vi "Pass data using reference.vi"(11 "error in":errorcluster) -> (15 "error out":errorcluster)   [LabVIEW 2021, in "Voltage Measurement.lvlib"]
uses:
  MeasurementCore/controls/Voltage Config.ctl
  MeasurementCore/controls/Current Config.ctl
  8c08564a-52c5-40b6-a610-6b453a234e3b.vi
  ff7b3996-5054-42a4-b452-886b26c0f36c.vi
  8c08564a-52c5-40b6-a610-6b453a234e3b.vi/36c45d0c-28c4-4d78-84df-ca3969178567.vi
  ff7b3996-5054-42a4-b452-886b26c0f36c.vi/36c45d0c-28c4-4d78-84df-ca3969178567.vi
  8c08564a-52c5-40b6-a610-6b453a234e3b.vi/36c45d0c-28c4-4d78-84df-ca3969178567.vi/6651a77e-856e-4bcd-af5a-c0c13b264cc1.vi
  ff7b3996-5054-42a4-b452-886b26c0f36c.vi/36c45d0c-28c4-4d78-84df-ca3969178567.vi/6651a77e-856e-4bcd-af5a-c0c13b264cc1.vi
  <vilib>/JDP Science/JSONtext/JSON text to Variant.vi
  <vilib>/JDP Science/JSONtext/LVClass Serializer/JSONtext LVClass Serializer.lvclass
  Voltage Measurement.lvlib
  MeasurementCore/Main_Voltage Measurement.lvlib
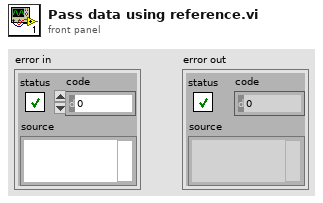
[diagram p1: front panel]
types:
  T1 = typedef "Main_Voltage Measurement.lvlib/Voltage Config.ctl" = cluster{"Voltage Level":dbl, "Voltage Level Range":dbl}
  T2 = typedef "Main_Voltage Measurement.lvlib/Current Config.ctl" = cluster{"Current Limit":dbl, "Current Limit Range":dbl}
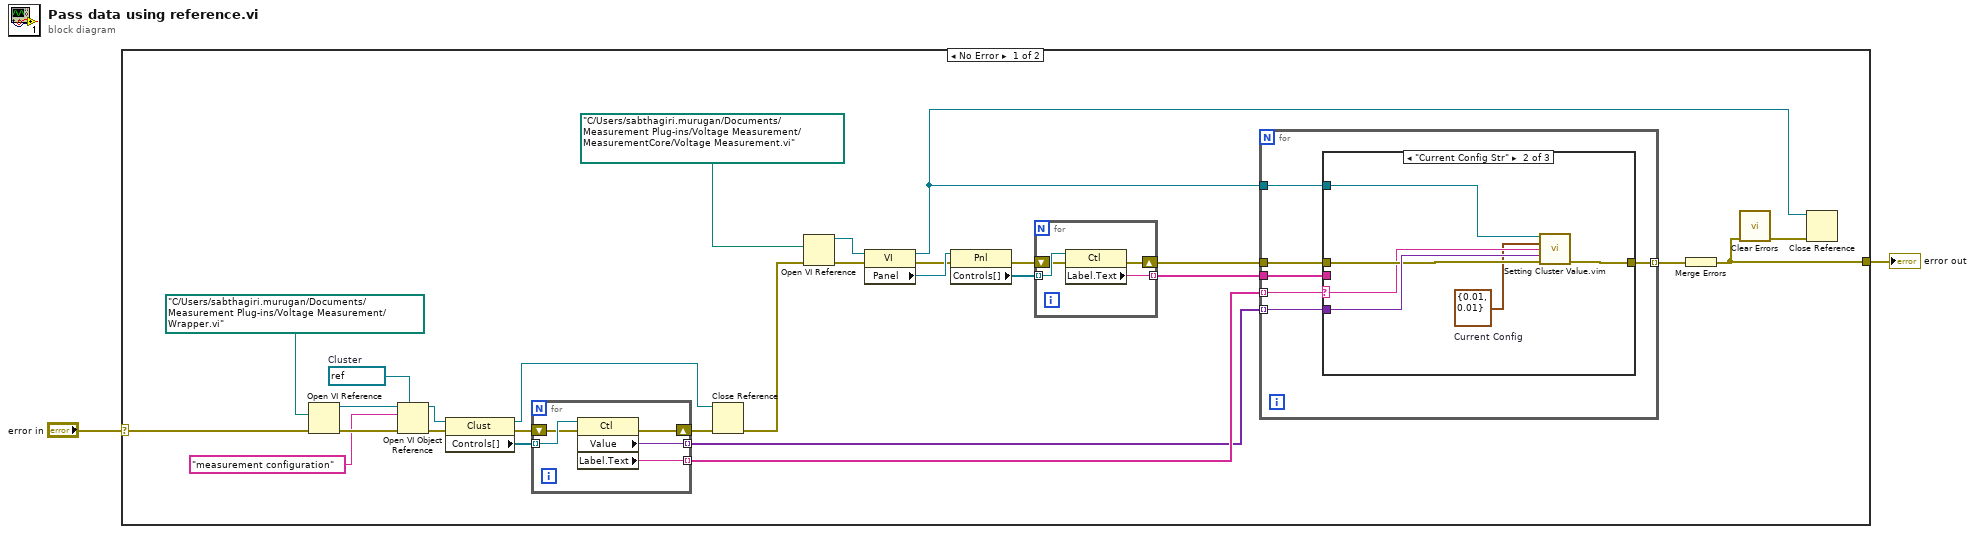
[diagram p0: block diagram]
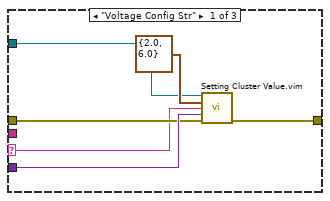
[diagram p2: hidden frame]
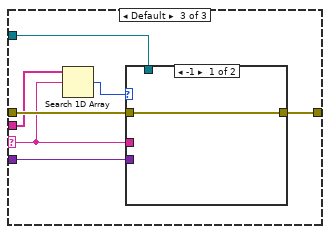
[diagram p3: hidden frame]
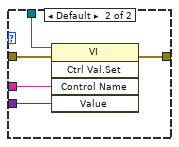
[diagram p4: hidden frame]
diagram:
  n1 = case shown="No Error" "error in" {
    selector: "error in" -> [w29 w71]
    tunnel: [w12 w71] -> w2
    frame No Error {
      w22 = refnum<vi> refnum  # Cluster
      n2 = Open VI Reference(vi path=path "C:/Users/sabthagiri.murugan/Documents/Measurement Plug-ins/Voltage Measurement/Wrapper.vi", error in (no error)=w29) -> (vi reference=w25:refnum<vi>, error out=w24:errorcluster)  [unwired: 4 in]
      n3 = Open VI Object Reference(7:w22, 8:w24, 10:"measurement configuration" ("Control Name"), 11:w25) -> (0:w20:errorcluster, 3:w21:refnum<vi>)
      n4 = property class="Clust"(reference=w21, error in=w20) -> (reference out=w13:refnum<vi>, error out=w18:errorcluster, "Controls[]"=w19:refnum<vi>[])
      n5 = for {
        tunnel: w19 -> [w39] mode=indexing
        shift-right: [w37] -> w15
        shift-left: w18 -> [w38]
        tunnel: [w36] -> w16 mode=indexing
        tunnel: [w35] -> w17 mode=indexing
        n6 = property class="Ctl"(reference=w39, error in=w38) -> (error out=w37:errorcluster, "Value"=w36:variant, "Label.Text"=w35:string)  [unwired: 1 out]
      }
      n7 = Close Reference(reference=w13, error in (no error)=w15) -> (error out=w14:errorcluster)
      n8 = Open VI Reference(vi path=path "C:/Users/sabthagiri.murugan/Documents/Measurement Plug-ins/Voltage Measurement/MeasurementCore/Voltage Measurement.vi", error in (no error)=w14) -> (vi reference=w10:refnum<vi>, error out=w28:errorcluster)  [unwired: 4 in]
      n9 = property class="VI"(reference=w10, error in=w28) -> (reference out=w9:refnum<vi>, error out=w7:errorcluster, "Panel"=w8:refnum<vi>)
      n10 = property class="Pnl"(reference=w8, error in=w7) -> (error out=w5:errorcluster, "Controls[]"=w6:refnum<vi>[])  [unwired: 1 out]
      n11 = for {
        tunnel: w6 -> [w34] mode=indexing
        shift-right: [w32] -> w4
        shift-left: w5 -> [w33]
        tunnel: [w31] -> w3 mode=indexing
        n12 = property class="Ctl"(reference=w34, error in=w33) -> (error out=w32:errorcluster, "Label.Text"=w31:string)  [unwired: 1 out]
      }
      n13 = for {
        tunnel: w9 -> [w45]
        tunnel: w4 -> [w44]
        tunnel: [w43] -> w26 mode=indexing
        tunnel: w17 -> [w42] mode=indexing
        tunnel: w16 -> [w41] mode=indexing
        tunnel: w3 -> [w40]
        n14 = case shown="\"Current Config Str\"" w42 {
          selector: w42 -> [w46 w53 w58]
          tunnel: w45 -> [w48 w55 w64]
          tunnel: w44 -> [w49 w56 w63]
          tunnel: [w47 w54 w62] -> w43
          tunnel: w41 -> [w51 w57 w61]
          tunnel: w40 -> [_ _ w60]
          frame "Voltage Config Str" {
            n15 = call "Setting Cluster Value.vim"("VI in"=w48, "Voltage Config"=T1 {"Voltage Level"=2.0, "Voltage Level Range"=6.0}, "String"=w46, "Value"=w51, "error in (no error)"=w49) -> ("error out"=w47:errorcluster)  [unwired: 10 in]
          }
          frame "Current Config Str" {
            w52 = T2 {"Current Limit"=0.01, "Current Limit Range"=0.01}  # Current Config
            n16 = call "Setting Cluster Value.vim"("VI in"=w55, "Voltage Config"=w52, "String"=w53, "Value"=w57, "error in (no error)"=w56) -> ("error out"=w54:errorcluster)  [unwired: 10 in]
          }
          frame Default {
            n17 = Search 1D Array(1D array=w60, element=w58) -> (index of element=w59:i32)  [unwired: 1 in]
            n18 = case shown="-1" w59 {
              tunnel: w64 -> [_ w70]
              tunnel: w63 -> [w65 w69]
              tunnel: [w65 w68] -> w62
              tunnel: w58 -> [_ w67]
              tunnel: w61 -> [_ w66]
              frame -1 {
              }
              frame Default {
                n19 = invoke class="VI" method="Ctrl Val.Set"(reference=w70, error in=w69, "Control Name"=w67, "Value"=w66) -> (error out=w68:errorcluster)  [unwired: 1 in, 4 out]
              }
            }
          }
        }
      }
      n20 = Merge Errors(w26) -> (w12:errorcluster)
      n21 = call <vilib>:"Clear Errors.vi"("error in (no error)"=w12) -> ("error out"=w11:errorcluster)  [unwired: 5 in, 1 out]
      n22 = Close Reference(reference=w9, error in (no error)=w11) -> ()  [unwired: 1 out]
    }
    frame Error {
    }
  }
  "error out" <- w2
